vi "ZM-ROOT-writePrelaunchSettings.vi"(8 "error in (no error)":errorcluster, 10 "settings":T1, 11 "ZM-ROOT-root in":refnum<class "ZM-ROOT-root.lvclass">) -> (0 "error out":errorcluster, 3 "ZM-ROOT-root out":refnum<class "ZM-ROOT-root.lvclass">)   [LabVIEW 2020, in "ZM-ROOT-root.lvlib" / "ZM-ROOT-root.lvclass"]
doc: "Public custom accessor: writes the pre-launch settings. The launcher fills ZM-ROOT-PRELAUNCH_SETTINGS (outputFolder, usePlaceholderHardware) and then launches the root."
uses:
  ZM-ROOT-root.lvclass
  ZM-ROOT-root.lvclass/ZM-ROOT-root.ctl
  ZM-ROOT-PRELAUNCH_SETTINGS.ctl
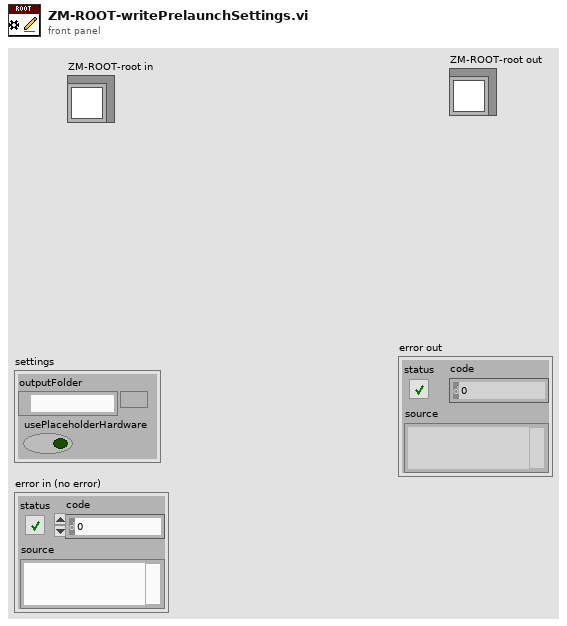
[diagram p1: front panel]
types:
  T1 = typedef "ZM-ROOT-root.lvlib/ZM-ROOT-root.lvclass/ZM-ROOT-PRELAUNCH_SETTINGS.ctl" = cluster{"outputFolder":path, "usePlaceholderHardware":bool}
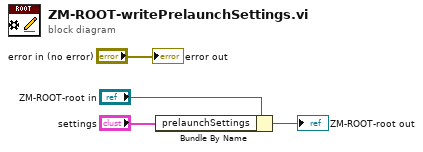
[diagram p0: block diagram]
diagram:
  n1 = Bundle By Name(cluster="ZM-ROOT-root in", "prelaunchSettings"="settings") -> (→"ZM-ROOT-root out":refnum<class "ZM-ROOT-root.lvclass">)
  "error out" <- "error in (no error)"
